vi "UDP UI.vi"() -> ()   [LabVIEW 2015, in "E2E Tag Exchange editor node.lvclass"]
uses:
  E2E Tag Exchange editor node.lvclass
  object references.ctl
  <vilib>/NI/DCAF/Tag Editor Core/Configuration Editor/Classes/Engine Parent/Engine Parent Editor Node.lvclass
  references.ctl
  <vilib>/NI/Configuration Framework/Node/StopEvent.ctl
  <vilib>/NI/Configuration Framework/Node/RefreshUIEvent.ctl
  <vilib>/NI/Configuration Framework/Node/CacheState.ctl
  <vilib>/NI/Configuration Framework/Node/NodeChangeEvent.ctl
  <vilib>/NI/Configuration Framework/Node/NodeRef.ctl
  <vilib>/NI/Configuration Framework/Node/NISE_CEF_Node.lvclass
  <vilib>/NI/AMC/Message Queue.ctl
  <vilib>/NI/AMC/Message.ctl
  <vilib>/NI/Tools/Keyed Array/KeyedArray.ctl
  UDP UI References.ctl
  <vilib>/NI/Tools/Keyed Array/Tools_KeyedArray.lvlib
  <vilib>/NI/AMC/AMC.lvlib
panel:
  in  "Estimated Array/String Size":i32 caption="Estimated Total Array/String Size (bytes)"
  in  "References":T1
  in  "node References":T7
  out "Estimated Output \nPacket Size (bytes)":i32
  out "Estimated Input \nPacket Size (bytes)":i32
  in  "Tag":string(combo)
  in  "Generate":bool
  in  "Last Update Tag?":bool
  out "local_Address":string="localhost" caption="Address"
  in  "input_Local Port":u16 caption="Local Port (read from)"
  in  "Remote Port":u16 caption="Remote Port (write to)"
  in  "output_Local Port":u16 caption="Local Port (write from)"
  in  "Address":string
  # "Output"
  # "Input"
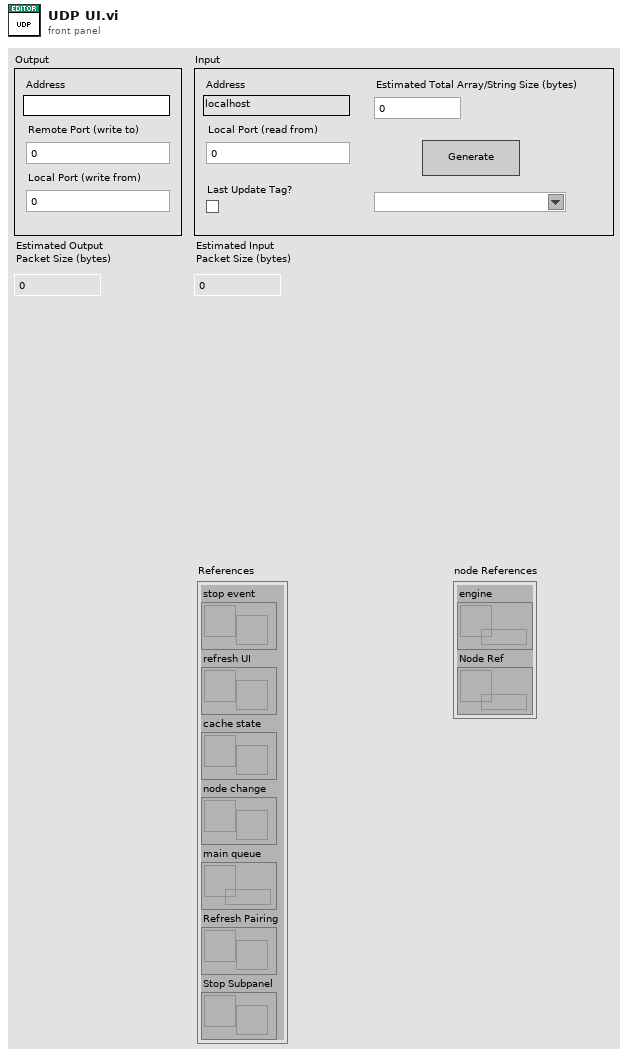
[diagram p1: front panel]
types:
  T1 = typedef "E2E Tag Exchange editor node.lvclass/references.ctl" = cluster{"stop event":T2, "refresh UI":T3, "cache state":T4, "node change":T5, "main queue":T6, "Refresh Pairing":refnum<user-event>, "Stop Subpanel":refnum<user-event>}
  T2 = typedef "NISE_CEF_Node.lvclass/StopEvent.ctl" = refnum<user-event>
  T3 = typedef "NISE_CEF_Node.lvclass/RefreshUIEvent.ctl" = refnum<user-event>
  T4 = typedef "NISE_CEF_Node.lvclass/CacheState.ctl" = refnum<user-event>
  T5 = typedef "NISE_CEF_Node.lvclass/NodeChangeEvent.ctl" = refnum<user-event>
  T6 = typedef "AMC.lvlib/Message Queue.ctl" = refnum<queue>
  T7 = typedef "E2E Tag Exchange editor node.lvclass/object references.ctl" = cluster{"engine":refnum<data-value>, "Node Ref":refnum<data-value>}
  T8 = typedef "E2E Tag Exchange editor node.lvclass/UDP UI References.ctl" = cluster{"Address":refnum<vi>, "Remote Port":refnum<vi>, "input_Local Port":refnum<vi>, "output_Local Port":refnum<vi>, "Last Update Tag?":refnum<vi>, "Tag":refnum<vi>, "Generate":refnum<vi>, "Input Packet Size":refnum<vi>, "Output Packet Size":refnum<vi>, "Estimated Array Size":refnum<vi>}
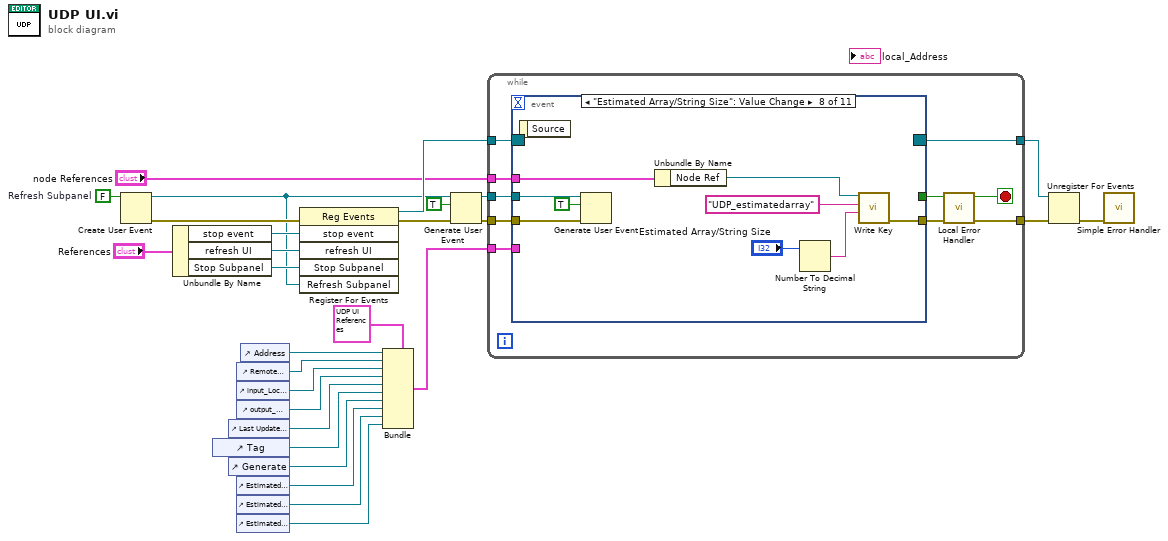
[diagram p0: block diagram]
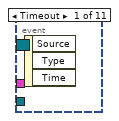
[diagram p2: hidden frame]
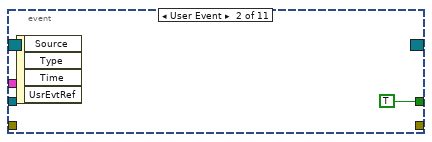
[diagram p3: hidden frame]
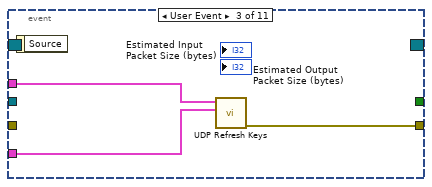
[diagram p4: hidden frame]
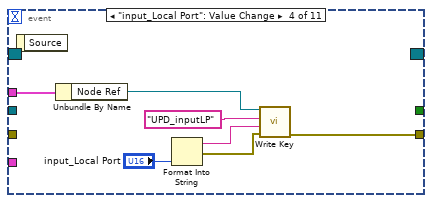
[diagram p5: hidden frame]
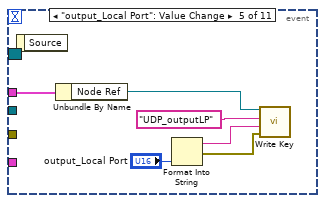
[diagram p6: hidden frame]
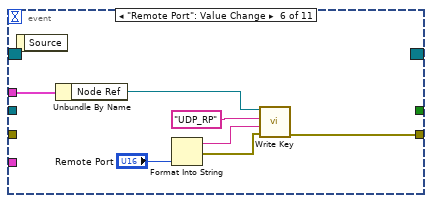
[diagram p7: hidden frame]
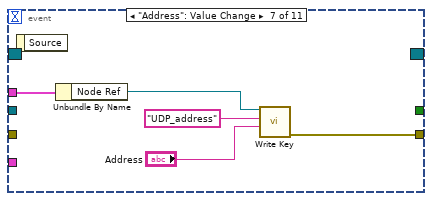
[diagram p8: hidden frame]
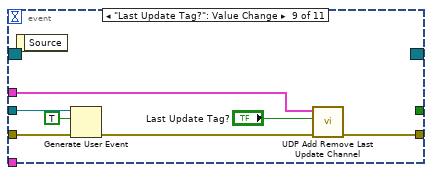
[diagram p9: hidden frame]
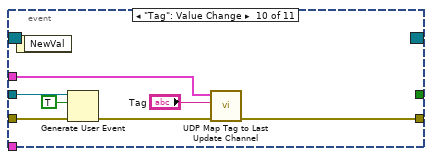
[diagram p10: hidden frame]
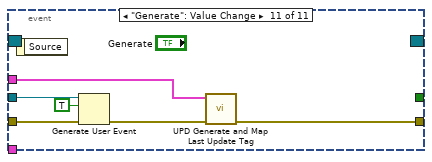
[diagram p11: hidden frame]
diagram:
  w22 = FALSE  # Refresh Subpanel
  n1 = Create User Event(user event datatype=w22) -> (user event=w2:refnum<user-event>, error out=w6:errorcluster)  [unwired: 1 in]
  n2 = Unbundle By Name("References") -> ("stop event"=w27:T2, "refresh UI"=w26:T3, "Stop Subpanel"=w25:refnum<user-event>)
  n3 = control-ref of="Tag"() -> (w15:refnum<vi>)
  n4 = control-ref of="Last Update Tag?"() -> (w16:refnum<vi>)
  n5 = control-ref of="Generate"() -> (w14:refnum<vi>)
  n6 = control-ref of="Remote Port"() -> (w19:refnum<vi>)
  n7 = control-ref of="input_Local Port"() -> (w18:refnum<vi>)
  n8 = control-ref of="output_Local Port"() -> (w17:refnum<vi>)
  n9 = control-ref of="Estimated Input \nPacket Size (bytes)"() -> (w12:refnum<vi>)
  n10 = control-ref of="Estimated Output \nPacket Size (bytes)"() -> (w11:refnum<vi>)
  n11 = control-ref of="Estimated Array/String Size"() -> (w1:refnum<vi>)
  n12 = control-ref of="Address"() -> (w20:refnum<vi>)
  n13 = register-events(error in=w6, w27, w26, w25, w2) -> (reference out=w24:refnum<event-registration>, error out=w5:errorcluster)  [unwired: 1 in]
  n14 = Bundle(cluster=T8 {"Address"=refnum, "Remote Port"=refnum, "input_Local Port"=refnum, "output_Local Port"=refnum, "Last Update Tag?"=refnum, "Tag"=refnum, "Generate"=refnum, "Input Packet Size"=refnum, "Output Packet Size"=refnum, "Estimated Array Size"=refnum} ("UDP UI References"), "Address"=w20, "Remote Port"=w19, "input_Local Port"=w18, "output_Local Port"=w17, "Last Update Tag?"=w16, "Tag"=w15, "Generate"=w14, "Input Packet Size"=w12, "Output Packet Size"=w11, "Estimated Array Size"=w1) -> (w13:T8)
  n15 = Generate User Event(user event=w2, event data cluster=TRUE ("event data"), error in=w5) -> (user event out=w3:refnum<user-event>, error out=w4:errorcluster)  [unwired: 1 in]
  n16 = while {
    tunnel: w24 -> [w38]
    tunnel: w4 -> [w37]
    tunnel: "node References" -> [w36]
    tunnel: w3 -> [w35]
    tunnel: w13 -> [w34]
    tunnel: [w30] -> w9
    tunnel: [w29] -> w8
    stop <- w32 stop-if-true
    n17 = event shown="[7] \"Estimated Array/String Size\": Value Change" {
      selector: w38 -> [_ _ _ _ _ _ _ _ _ _ _]
      dyn-events: [_ _ _ _ _ _ _ _ _ _ _] -> w30
      timeout: _ -> [_ _ _ _ _ _ _ _ _ _ _]
      tunnel: w37 -> [_ _ _ _ _ _ _ w69 w78 w86 w92]
      tunnel: [_ TRUE _ _ _ _ _ _ _ _ _] -> w31
      tunnel: w36 -> [_ _ w40 w49 w55 w62 w67 w76 w82 w89 w96]
      tunnel: [_ _ w42 w43 _ w56 w64 w73 w83 w90 w95] -> w33
      tunnel: w35 -> [_ _ _ _ _ _ _ w68 w79 w85 w93]
      tunnel: w34 -> [_ _ w41 _ _ _ _ _ _ _ _]
      event Timeout {
        n18 = event-data() -> ()  [unwired: 1 in, 3 out]
      }
      event User Event {
        n19 = event-data() -> ()  [unwired: 1 in, 4 out]
      }
      event User Event {
        n20 = event-data() -> ()  [unwired: 1 in, 1 out]
        n21 = call "UDP Refresh Keys.vi"("UDP UI References"=w41, "node References"=w40) -> ("error out"=w42:errorcluster)  [unwired: 7 in, 2 out]
      }
      event "input_Local Port": Value Change {
        n22 = event-data() -> ()  [unwired: 1 in, 1 out]
        n23 = Unbundle By Name(w49) -> ("Node Ref"=w48:refnum<data-value>)
        n24 = Format Into String("input_Local Port") -> (resulting string=w46:string, error out=w45:errorcluster)  [unwired: 3 in]
        n25 = call "Write Key.vi"("error in (no error)"=w45, "Value"=w46, "Key"="UPD_inputLP", "E2E editor node in"=w48) -> ("error out"=w43:errorcluster)  [unwired: 6 in, 1 out]
      }
      event "output_Local Port": Value Change {
        n26 = event-data() -> ()  [unwired: 1 in, 1 out]
        n27 = Unbundle By Name(w55) -> ("Node Ref"=w54:refnum<data-value>)
        n28 = Format Into String("output_Local Port") -> (resulting string=w53:string, error out=w52:errorcluster)  [unwired: 3 in]
        n29 = call "Write Key.vi"("error in (no error)"=w52, "Value"=w53, "Key"="UDP_outputLP", "E2E editor node in"=w54) -> ()  [unwired: 6 in, 2 out]
      }
      event "Remote Port": Value Change {
        n30 = event-data() -> ()  [unwired: 1 in, 1 out]
        n31 = Unbundle By Name(w62) -> ("Node Ref"=w61:refnum<data-value>)
        n32 = Format Into String("Remote Port") -> (resulting string=w60:string, error out=w59:errorcluster)  [unwired: 3 in]
        n33 = call "Write Key.vi"("error in (no error)"=w59, "Value"=w60, "Key"="UDP_RP", "E2E editor node in"=w61) -> ("error out"=w56:errorcluster)  [unwired: 6 in, 1 out]
      }
      event "Address": Value Change {
        n34 = event-data() -> ()  [unwired: 1 in, 1 out]
        n35 = Unbundle By Name(w67) -> ("Node Ref"=w66:refnum<data-value>)
        n36 = call "Write Key.vi"("Value"="Address", "Key"="UDP_address", "E2E editor node in"=w66) -> ("error out"=w64:errorcluster)  [unwired: 7 in, 1 out]
      }
      event "Estimated Array/String Size": Value Change {
        n37 = event-data() -> ()  [unwired: 1 in, 1 out]
        n38 = Generate User Event(user event=w68, event data cluster=TRUE, error in=w69) -> ()  [unwired: 1 in, 2 out]
        n39 = Unbundle By Name(w76) -> ("Node Ref"=w75:refnum<data-value>)
        n40 = Number To Decimal String(number="Estimated Array/String Size") -> (decimal integer string=w71:string)  [unwired: 1 in]
        n41 = call "Write Key.vi"("Value"=w71, "Key"="UDP_estimatedarray", "E2E editor node in"=w75) -> ("error out"=w73:errorcluster)  [unwired: 7 in, 1 out]
      }
      event "Last Update Tag?": Value Change {
        n42 = event-data() -> ()  [unwired: 1 in, 1 out]
        n43 = Generate User Event(user event=w79, event data cluster=TRUE, error in=w78) -> (error out=w77:errorcluster)  [unwired: 1 in, 1 out]
        n44 = call "UDP Add Remove Last Update Channel.vi"("error in (no error)"=w77, "Last Update Tag?"="Last Update Tag?", "node References"=w82) -> ("error out"=w83:errorcluster)  [unwired: 7 in, 1 out]
      }
      event "Tag": Value Change {
        n45 = event-data() -> ()  [unwired: 1 in, 1 out]
        n46 = Generate User Event(user event=w85, event data cluster=TRUE, error in=w86) -> (error out=w84:errorcluster)  [unwired: 1 in, 1 out]
        n47 = call "UDP Map Tag to Last Update Channel.vi"("error in (no error)"=w84, "Tag Name"="Tag", "node References"=w89) -> ("error out"=w90:errorcluster)  [unwired: 7 in, 1 out]
      }
      event "Generate": Value Change {
        n48 = event-data() -> ()  [unwired: 1 in, 1 out]
        n49 = Generate User Event(user event=w93, event data cluster=TRUE ("event data"), error in=w92) -> (error out=w91:errorcluster)  [unwired: 1 in, 1 out]
        n50 = call "UPD Generate and Map Last Update Tag.vi"("error in (no error)"=w91, "node References"=w96) -> ("error out"=w95:errorcluster)  [unwired: 8 in, 1 out]
      }
    }
    n51 = call "Local Error Handler.vi"("error in"=w33, "Stop in"=w31) -> ("error out"=w29:errorcluster, "Stop out"=w32:bool)  [unwired: 8 in]
  }
  n52 = Unregister For Events(event registration refnum=w9, error in=w8) -> (error out=w7:errorcluster)
  n53 = call <vilib>:"Simple Error Handler.vi"("error in (no error)"=w7) -> ()  [unwired: 4 in, 5 out]
